vi "Raise Required Override Error.vi"(0 "RFFE Command in":refnum<class "RFFE Command.lvclass">, 5 "VI Refnum in (This VI)":refnum<vi>, 11 "error in (no error)":errorcluster) -> (4 "RFFE Command out":refnum<class "RFFE Command.lvclass">, 6 "VI Refnum out":refnum<vi>, 15 "error out":errorcluster)   [LabVIEW 2018, in "MIPI RFFE API.lvlib" / "RFFE Command.lvclass"]
uses:
  RFFE Command.lvclass
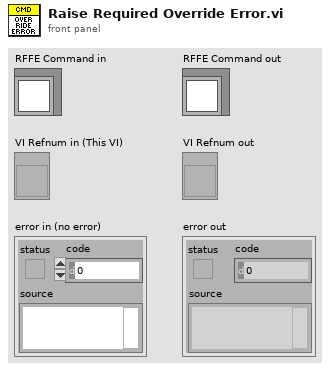
[diagram p1: front panel]
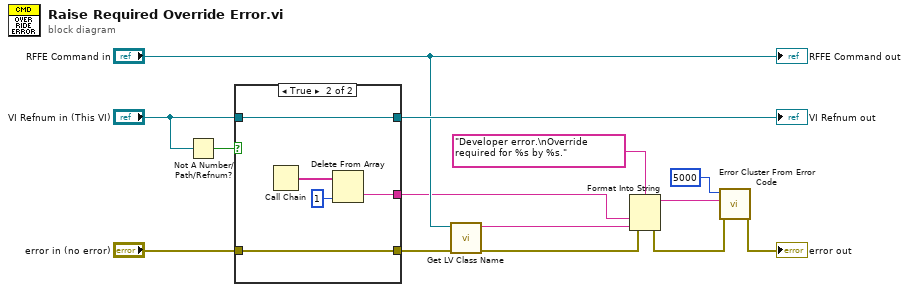
[diagram p0: block diagram]
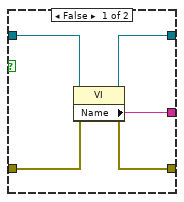
[diagram p2: hidden frame]
diagram:
  n1 = Not A Number/Path/Refnum?(number/path/refnum="VI Refnum in (This VI)") -> (NaN/Path/Refnum?=w5:bool)
  n2 = case shown="True" w5 {
    tunnel: "VI Refnum in (This VI)" -> [w16 w24]
    tunnel: "error in (no error)" -> [w19 w22]
    tunnel: [w15 w23] -> w4
    tunnel: [w18 w22] -> w3
    tunnel: [w17 w24] -> w11
    frame False {
      n3 = property class="VI"(reference=w16, error in=w19) -> (reference out=w17:refnum<vi>, error out=w18:errorcluster, "Name"=w15:string)
    }
    frame True {
      n4 = Call Chain() -> (call chain=w21:string[])
      n5 = Delete From Array(array=w21, index=1) -> (deleted portion=w23:string)  [unwired: 1 in, 1 out]
    }
  }
  "VI Refnum out" <- w11
  n6 = call <vilib>:"Get LV Class Name.vi"("error in (no error)"=w3, "object"="RFFE Command in") -> ("error out"=w2:errorcluster, "class name"=w1:string)  [unwired: 8 in]
  n7 = Format Into String(format string="Developer error.\nOverride required for %s by %s.", error in=w2, w4, w1) -> (resulting string=w7:string, error out=w6:errorcluster)  [unwired: 1 in]
  n8 = call <vilib>:"Error Cluster From Error Code.vi"("error in (no error)"=w6, "error message (\"\")"=w7, "error code (0)"=5000) -> ("error out"=→"error out":errorcluster)  [unwired: 6 in]
  "RFFE Command out" <- "RFFE Command in"
